vi "Result Comparison.vi"(0 "input cluster":T4={"User name"="COM1", "user account"="COM1", "UI"=[], "DI"=[], "Barcode"="", "MCListbox Ref_in"=refnum, "sequence step #"=0, "Result?"=FALSE, "Report Path"=path "", "Test Sequence"=enum."Initialization", "skip Test  "=[FALSE, FALSE, FALSE, FALSE, FALSE, FALSE, FALSE, FALSE, FALSE, FALSE, FALSE, FALSE, FALSE, FALSE, FALSE, FALSE, FALSE, FALSE, FALSE, FALSE, FALSE, FALSE, FALSE, FALSE, FALSE, FALSE, FALSE, FALSE, FALSE, FALSE, FALSE, FALSE]} {"DI"."Upper limit" format="%#_7f"; "DI"."Lower limit" format="%#_7f"}, 5 "measured data":dbl format="%#_13g", 9 "Measued String":string, 11 "error in (no error)":errorcluster) -> (4 "Output cluster":T4={"User name"="COM1", "user account"="COM1", "UI"=[], "DI"=[], "Barcode"="", "MCListbox Ref_in"=refnum, "sequence step #"=0, "Result?"=FALSE, "Report Path"=path "", "Test Sequence"=enum."Initialization", "skip Test  "=[FALSE, FALSE, FALSE, FALSE, FALSE, FALSE, FALSE, FALSE, FALSE, FALSE, FALSE, FALSE, FALSE, FALSE, FALSE, FALSE, FALSE, FALSE, FALSE, FALSE, FALSE, FALSE, FALSE, FALSE, FALSE, FALSE, FALSE, FALSE, FALSE, FALSE, FALSE, FALSE]} {"DI"."Upper limit" format="%#_7f"; "DI"."Lower limit" format="%#_7f"}, 6 "result":string, 8 "measured value":string, 10 "result?":bool, 15 "error out":errorcluster)   [LabVIEW 2021]
uses:
  5.ACTIVITIES/1.LabVIEW_State_Machine_Template/LabVIEW_State_Machine_Template/LabVIEW_State_Machine_Template/Project_Template/Queue Test updator/Controls/initialise cluster.ctl
  5.ACTIVITIES/1.LabVIEW_State_Machine_Template/LabVIEW_State_Machine_Template/LabVIEW_State_Machine_Template/Project_Template/Queue Test updator/Controls/test step description.ctl
  5.ACTIVITIES/1.LabVIEW_State_Machine_Template/LabVIEW_State_Machine_Template/LabVIEW_State_Machine_Template/Project_Template/Queue Test updator/Controls/comparison selection.ctl
  controls/Main test sequence.ctl
panel:
  out "Main test sequence":T1
  out "DI":T2[](array[typedef]) {"Upper limit" format="%#_7f"; "Lower limit" format="%#_7f"}
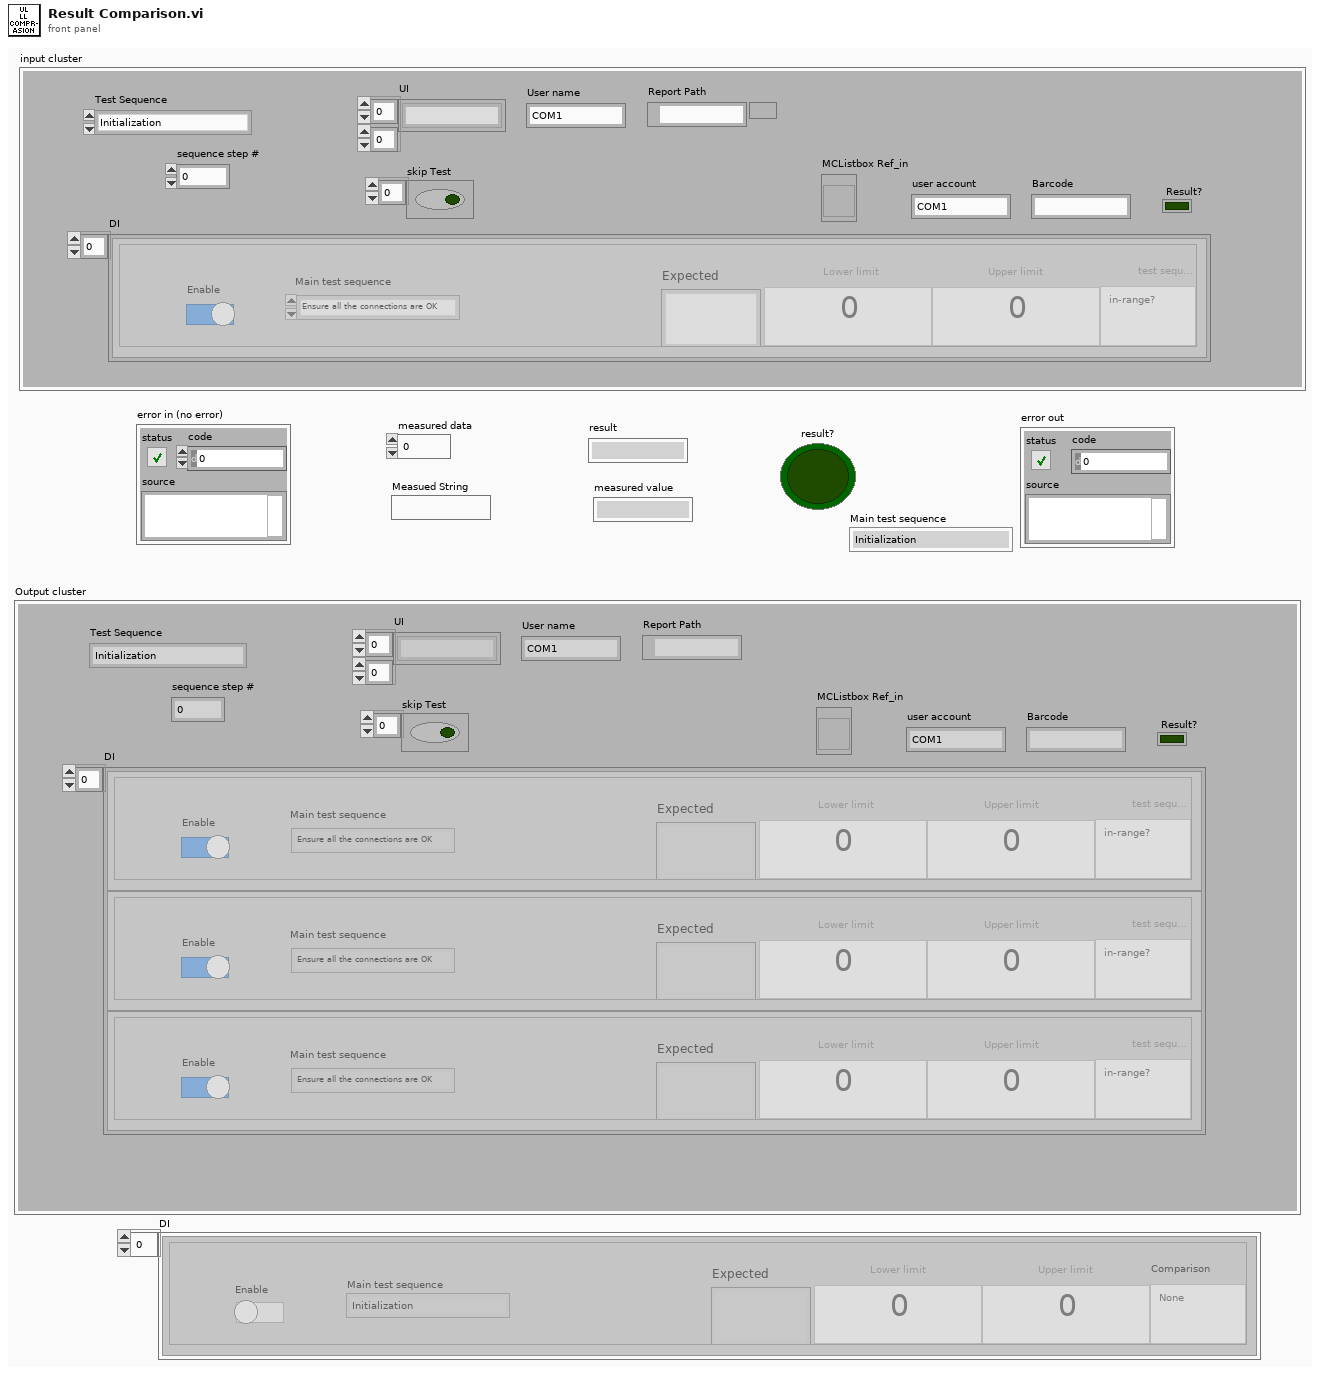
[diagram p1: front panel]
types:
  T1 = typedef "Main test sequence.ctl" = enum16{"Initialization", "Ensure all the connections are OK", "Turn ON 230V AC Input", "Load the Firmware", "Unlock_Opensesame & Stop console Logs", "Earth Detection", "Read Firmware", "Read & Write PCB Serial No", "Emergancy Switch Check", "Update WIFI credentials ", "Reboot", "Unlock Opensesame & Stop_console Logs", "WIFI State", "WIFI SSID", "Board revision", "ADC NTC Temp", "ADC_TYPE2_RCD_CURRENT", "5V Output Voltage", "3.3V Output Voltage", "D+M Sense", "Output Weld Sense", "FW Power Reset", "Unlock Opensesame & Stop console_Logs", "Reset switch Check", "Exit"}
  T2 = typedef "test step description.ctl" = cluster{"Lower limit":dbl, "Upper limit":dbl, "Comparison":T3, "Expected":string, "Enable":bool, "Main test sequence":T1}
  T3 = typedef "comparison selection.ctl" = enum16{"None", "in-range?", "less than?", "greater than?", "equal to?", "not equal to?", "less or equal to?", "greater or equal to?"}
  T4 = typedef "initialise cluster.ctl" = cluster{"User name":string, "user account":string, "UI":string[][], "DI":T2[], "Barcode":string, "MCListbox Ref_in":refnum<vi>, "sequence step #":u32, "Result?":bool, "Report Path":path, "Test Sequence":T1, "skip Test  ":bool[]}
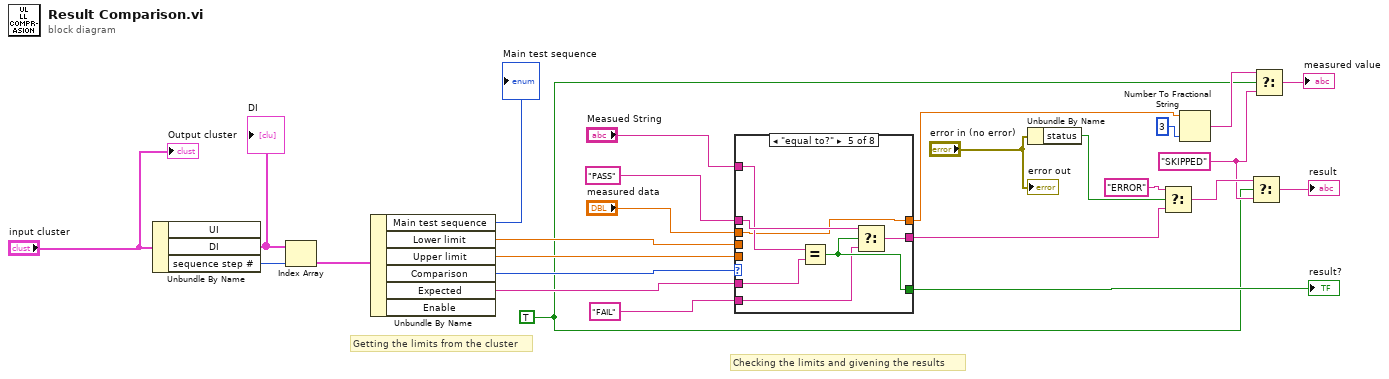
[diagram p0: block diagram]
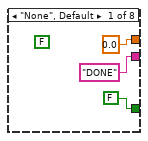
[diagram p2: hidden frame]
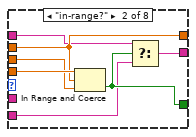
[diagram p3: hidden frame]
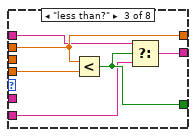
[diagram p4: hidden frame]
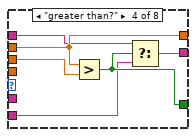
[diagram p5: hidden frame]
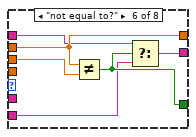
[diagram p6: hidden frame]
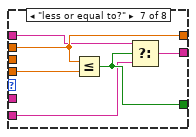
[diagram p7: hidden frame]
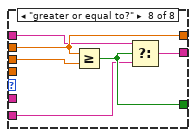
[diagram p8: hidden frame]
diagram:
  w3 = TRUE ("s")
  w6 = "SKIPPED" ("f")
  # "Checking the limits and givening the results"
  # "Getting the limits from the cluster"
  n1 = Unbundle By Name("input cluster") -> ("DI"=w25:T2[], "sequence step #"=w1:u32)  [unwired: 1 out]
  "DI" <- w25
  n2 = Index Array(array=w25, index=w1) -> (element=w24:T2)
  n3 = Unbundle By Name(w24) -> ("Main test sequence"=→"Main test sequence":T1, "Lower limit"=w11:dbl, "Upper limit"=w10:dbl, "Comparison"=w12:T3, "Expected"=w9:string)  [unwired: 1 out]
  n4 = case shown="\"equal to?\"" w12 {
    tunnel: ["DONE" ("f") w34 w42 w47 w55 w60 w67 w72] -> w19
    tunnel: w10 -> [_ w36 w37 _ _ _ w62 _]
    tunnel: w11 -> [_ w35 _ w48 _ w61 _ w73]
    tunnel: "measured data" -> [_ w32 w40 w45 w49 w58 w65 w70]
    tunnel: [FALSE w33 w41 w46 w54 w59 w66 w71] -> w4
    tunnel: [0.0 ("Measured Data") w32 w40 w45 w49 w58 w65 w70] -> w18
    tunnel: "PASS" ("t") -> [_ w31 w39 w43 w53 w57 w64 w69]
    tunnel: "FAIL" ("f") -> [_ w30 w38 w44 w52 w56 w63 w68]
    tunnel: w9 -> [_ _ _ _ w51 _ _ _]
    tunnel: "Measued String" -> [_ _ _ _ w50 _ _ _]
    frame "None", Default {
      (unwired) FALSE
    }
    frame "in-range?" {
      n5 = In Range and Coerce(upper limit=w36, x=w32, lower limit=w35) -> (In Range?=w33:bool)  [unwired: 1 out]
      n6 = Select(t=w31, s=w33, f=w30) -> (s? t:f=w34:string)
    }
    frame "less than?" {
      n7 = Less?(x=w40, y=w37) -> (x < y?=w41:bool)
      n8 = Select(t=w39, s=w41, f=w38) -> (s? t:f=w42:string)
    }
    frame "greater than?" {
      n9 = Greater?(x=w45, y=w48) -> (0:w46:bool)
      n10 = Select(t=w43, s=w46, f=w44) -> (s? t:f=w47:string)
    }
    frame "equal to?" {
      n11 = Equal?(x=w50, y=w51) -> (x = y?=w54:bool)
      n12 = Select(t=w53, s=w54, f=w52) -> (s? t:f=w55:string)
    }
    frame "not equal to?" {
      n13 = Not Equal?(x=w58, y=w61) -> (x != y?=w59:bool)
      n14 = Select(t=w57, s=w59, f=w56) -> (s? t:f=w60:string)
    }
    frame "less or equal to?" {
      n15 = Less Or Equal?(x=w65, y=w62) -> (x <= y?=w66:bool)
      n16 = Select(t=w64, s=w66, f=w63) -> (s? t:f=w67:string)
    }
    frame "greater or equal to?" {
      n17 = Greater Or Equal?(x=w70, y=w73) -> (x >= y?=w71:bool)
      n18 = Select(t=w69, s=w71, f=w68) -> (s? t:f=w72:string)
    }
  }
  "result?" <- w4
  n19 = Unbundle By Name("error in (no error)") -> ("status"=w21:bool)
  n20 = Select(t="ERROR" ("message"), s=w21, f=w19) -> (s? t:f=w7:string)
  n21 = Number To Fractional String(number=w18, precision (6)=i16 3) -> (F-format string=w5:string)  [unwired: 2 in]
  n22 = Select(t=w7, s=w3, f=w6) -> (s? t:f=→"result":string)
  n23 = Select(t=w5, s=w3, f=w6) -> (s? t:f=→"measured value":string)
  "error out" <- "error in (no error)"
  "Output cluster" <- "input cluster"
